vi "Process Feedback.vi"(8 "error in":errorcluster, 10 "Channel Feedback":T1, 11 "Sequence Executor in":refnum<class "Sequence Executor.lvclass">) -> (0 "error out":errorcluster, 3 "Sequence Executor out":refnum<class "Sequence Executor.lvclass">)   [LabVIEW 2026, in "Sequence Executor.lvclass"]
doc: "Handles one Channel Feedback from the rig. Stores Last Feedback; writes the Channel Values display (2-D string name | value | unit); if Running: latch Step Start ms on first feedback, Evaluate Step, and on done record the result and advance (Begin Step) or Finish Sequence."
uses:
  Sequence Executor.lvclass
  Sequence Executor.lvclass/Sequence Executor.ctl
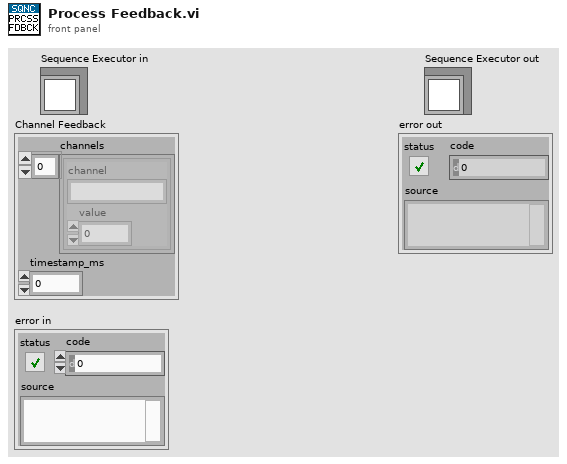
[diagram p1: front panel]
types:
  T1 = cluster{"channels":cluster{"channel":string, "value":dbl}[], "timestamp_ms":dbl}
  T2 = cluster{"step_no":i32, "step_name":string, "result":string, "reason":string, "measured":dbl, "target":dbl, "duration_ms":dbl}
  T3 = typedef "Rig Config.ctl" = cluster{"rig_id":string, "description":string, "plugin_class":string, "channels":T4[]}
  T4 = typedef "Channel Definition.ctl" = cluster{"name":string, "unit":string, "min":dbl, "max":dbl}
  T5 = typedef "Step Phase.ctl" = enum16{"Idle", "Settling", "Dwell", "Complete"}
  T6 = typedef "Sequence File.ctl" = cluster{"sequence_id":string, "description":string, "rig_config":string, "steps":T7[]}
  T7 = typedef "Step Config.ctl" = cluster{"step_no":i32, "step_name":string, "command_type":string, "setpoints":T8[], "conditions":T9[], "dwell_time_ms":i32, "timeout_ms":i32, "expected_result":string}
  T8 = typedef "Channel Value.ctl" = cluster{"channel":string, "value":dbl}
  T9 = typedef "Condition.ctl" = cluster{"channel":string, "target":dbl, "tolerance":dbl}
  T10 = typedef "Step Result.ctl" = cluster{"step_no":i32, "step_name":string, "result":string, "reason":string, "measured":dbl, "target":dbl, "duration_ms":dbl}
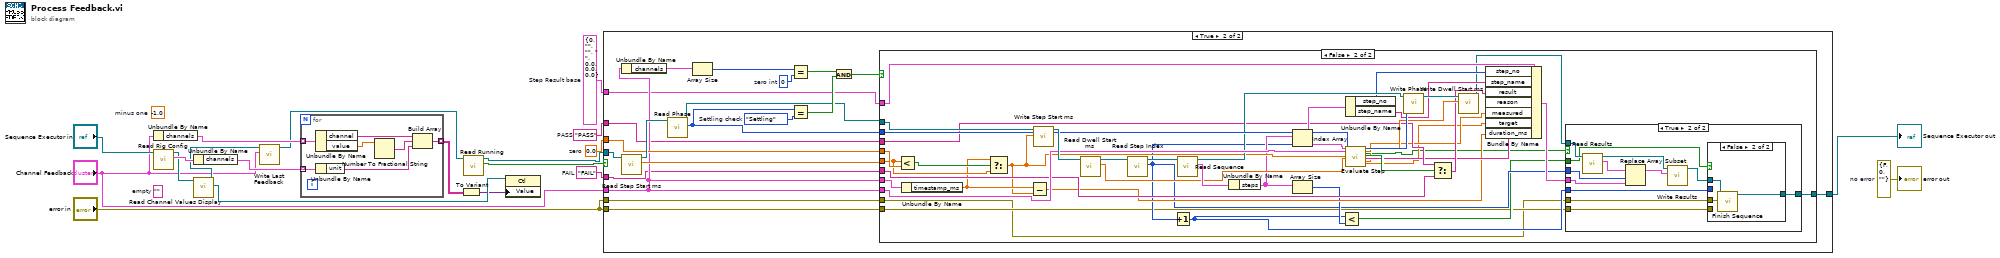
[diagram p0: block diagram]
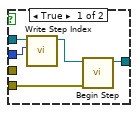
[diagram p5: hidden frame]
diagram:
  (unwired) -1.0  # minus one
  (unwired) ""  # empty
  w5 = T2 {"step_no"=0, "step_name"="", "result"="", "reason"=" ", "measured"=0.0, "target"=0.0, "duration_ms"=0.0}  # Step Result base
  w6 = "FAIL"  # FAIL
  w7 = "PASS"  # PASS
  w8 = 0.0  # zero
  w1 = errorcluster {"status"=FALSE, "code"=0, "source"=""}  # no error
  n1 = Unbundle By Name("Channel Feedback") -> ("channels"=w18:cluster{"channel":string, "value":dbl}[])
  n2 = call "Read Rig Config.vi"("Sequence Executor in"="Sequence Executor in") -> ("Rig Config"=w19:T3, "Sequence Executor out"=w16:refnum<class "Sequence Executor.lvclass">)  [unwired: 8 in, 1 out]
  n3 = Unbundle By Name(w19) -> ("channels"=w17:T4[])
  n4 = call "Read Channel Values Display.vi"("Sequence Executor in"=w16) -> ("Channel Values Display"=w14:refnum<vi>, "Sequence Executor out"=w12:refnum<class "Sequence Executor.lvclass">)  [unwired: 8 in, 1 out]
  n5 = call "Write Last Feedback.vi"("Channel Feedback"="Channel Feedback", "Sequence Executor in"=w12) -> ("Sequence Executor out"=w11:refnum<class "Sequence Executor.lvclass">)  [unwired: 8 in, 1 out]
  n6 = for {
    tunnel: w18 -> [w27] mode=indexing
    tunnel: w17 -> [w25] mode=indexing
    tunnel: [w21] -> w15 mode=indexing
    n7 = Unbundle By Name(w27) -> ("channel"=w24:string, "value"=w26:dbl)
    n8 = Unbundle By Name(w25) -> ("unit"=w22:string)
    n9 = Number To Fractional String(number=w26) -> (F-format string=w23:string)  [unwired: 3 in]
    n10 = Build Array(w24, w23, w22) -> (w21:string[])
  }
  n11 = To Variant(anything=w15) -> (Variant=w13:variant)
  n12 = call "Read Running.vi"("Sequence Executor in"=w11) -> ("Running"=w3:bool, "Sequence Executor out"=w10:refnum<class "Sequence Executor.lvclass">)  [unwired: 8 in, 1 out]
  n13 = property class="Ctl"(reference=w14, "Value"=w13) -> ()  [unwired: 1 in, 2 out]
  n14 = case shown="True" w3 {
    tunnel: w10 -> [w28 w48]
    tunnel: "Channel Feedback" -> [_ w36]
    tunnel: [w28 w29] -> w2
    tunnel: w8 -> [_ w37]
    tunnel: w7 -> [_ w35]
    tunnel: w6 -> [_ w34]
    tunnel: w5 -> [_ w33]
    tunnel: "error in" -> [_ w32]
    tunnel: "error in" -> [_ w31]
    frame False {
    }
    frame True {
      w43 = enum16{"Idle", "Settling", "Dwell", "Complete"}."Settling"  # Settling check
      w44 = 0  # zero int
      n15 = Unbundle By Name(w36) -> ("channels"=w46:cluster{"channel":string, "value":dbl}[])
      n16 = call "Read Step Start ms.vi"("Sequence Executor in"=w48) -> ("Step Start ms"=w39:dbl, "Sequence Executor out"=w47:refnum<class "Sequence Executor.lvclass">)  [unwired: 8 in, 1 out]
      n17 = call "Read Phase.vi"("Sequence Executor in"=w47) -> ("Step Phase"=w38:T5, "Sequence Executor out"=w40:refnum<class "Sequence Executor.lvclass">)  [unwired: 8 in, 1 out]
      n18 = Array Size(array=w46) -> (size(s)=w45:i32)
      n19 = Equal?(x=w45, y=w44) -> (x = y?=w42:bool)
      n20 = Equal?(x=w38, y=w43) -> (x = y?=w41:bool)
      n21 = And(x=w42, y=w41) -> (x .and. y?=w30:bool)
      n22 = case shown="False" w30 {
        tunnel: w40 -> [w49 w86]
        tunnel: w39 -> [_ w87]
        tunnel: w36 -> [_ w89]
        tunnel: w38 -> [_ w80]
        tunnel: [w49 w50] -> w29
        tunnel: w37 -> [_ w90]
        tunnel: w36 -> [_ w81]
        tunnel: w35 -> [_ w73]
        tunnel: w34 -> [_ w71]
        tunnel: w33 -> [_ w61]
        tunnel: w32 -> [_ w53]
        tunnel: w31 -> [_ w52]
        frame True {
        }
        frame False {
          n23 = Less?(x=w87, y=w90) -> (x < y?=w88:bool)
          n24 = Unbundle By Name(w89) -> ("timestamp_ms"=w70:dbl)
          n25 = Select(t=w70, s=w88, f=w87) -> (s? t:f=w69:dbl)
          n26 = Subtract(x=w70, y=w69) -> (x-y=w62:dbl)
          n27 = call "Write Step Start ms.vi"("Step Start ms"=w69, "Sequence Executor in"=w86) -> ("Sequence Executor out"=w85:refnum<class "Sequence Executor.lvclass">)  [unwired: 8 in, 1 out]
          n28 = call "Read Dwell Start ms.vi"("Sequence Executor in"=w85) -> ("Dwell Start ms"=w79:dbl, "Sequence Executor out"=w84:refnum<class "Sequence Executor.lvclass">)  [unwired: 8 in, 1 out]
          n29 = call "Read Step Index.vi"("Sequence Executor in"=w84) -> ("Step Index"=w56:i32, "Sequence Executor out"=w83:refnum<class "Sequence Executor.lvclass">)  [unwired: 8 in, 1 out]
          n30 = Increment(x=w56) -> (x+1=w55:i32)
          n31 = call "Read Sequence.vi"("Sequence Executor in"=w83) -> ("Sequence File"=w82:T6, "Sequence Executor out"=w78:refnum<class "Sequence Executor.lvclass">)  [unwired: 8 in, 1 out]
          n32 = Unbundle By Name(w82) -> ("steps"=w60:T7[])
          n33 = Index Array(array=w60, index=w56) -> (element=w74:T7)
          n34 = Array Size(array=w60) -> (size(s)=w59:i32)
          n35 = Less?(x=w55, y=w59) -> (x < y?=w54:bool)
          n36 = Unbundle By Name(w74) -> ("step_no"=w68:i32, "step_name"=w67:string)
          n37 = call "Evaluate Step.vi"("Step Config"=w74, "Channel Feedback"=w81, "Step Phase in"=w80, "step start ms"=w69, "dwell start ms"=w79) -> ("Step Phase out"=w77:T5, "dwell start ms out"=w75:dbl, "done"=w51:bool, "passed"=w72:bool, "reason"=w65:string, "measured"=w64:dbl, "target"=w63:dbl)  [unwired: 16 in]
          n38 = call "Write Phase.vi"("Step Phase"=w77, "Sequence Executor in"=w78) -> ("Sequence Executor out"=w76:refnum<class "Sequence Executor.lvclass">)  [unwired: 8 in, 1 out]
          n39 = Select(t=w73, s=w72, f=w71) -> (s? t:f=w66:string)
          n40 = call "Write Dwell Start ms.vi"("Dwell Start ms"=w75, "Sequence Executor in"=w76) -> ("Sequence Executor out"=w58:refnum<class "Sequence Executor.lvclass">)  [unwired: 8 in, 1 out]
          n41 = Bundle By Name(cluster=w61, "step_no"=w68, "step_name"=w67, "result"=w66, "reason"=w65, "measured"=w64, "target"=w63, "duration_ms"=w62) -> (w57:T2)
          n42 = case shown="True" w51 {
            tunnel: w58 -> [w91 w103]
            tunnel: w57 -> [_ w100]
            tunnel: w56 -> [_ w101]
            tunnel: w55 -> [_ w96]
            tunnel: w54 -> [_ w93]
            tunnel: [w91 w92] -> w50
            tunnel: w53 -> [_ w95]
            tunnel: w52 -> [_ w94]
            frame False {
            }
            frame True {
              n43 = call "Read Results.vi"("Sequence Executor in"=w103) -> ("Results"=w102:T10[], "Sequence Executor out"=w99:refnum<class "Sequence Executor.lvclass">)  [unwired: 8 in, 1 out]
              n44 = Replace Array Subset(array=w102, new element=w100, index=w101) -> (w98:T10[])
              n45 = call "Write Results.vi"("Results"=w98, "Sequence Executor in"=w99) -> ("Sequence Executor out"=w97:refnum<class "Sequence Executor.lvclass">)  [unwired: 8 in, 1 out]
              n46 = case shown="False" w93 {
                tunnel: w97 -> [w108 w111]
                tunnel: w96 -> [w107 _]
                tunnel: w95 -> [w105 _]
                tunnel: [w104 w109] -> w92
                tunnel: w94 -> [_ w110]
                frame True {
                  n47 = call "Write Step Index.vi"("Step Index"=w107, "Sequence Executor in"=w108) -> ("Sequence Executor out"=w106:refnum<class "Sequence Executor.lvclass">)  [unwired: 8 in, 1 out]
                  n48 = call "Begin Step.vi"("error in"=w105, "Sequence Executor in"=w106) -> ("Sequence Executor out"=w104:refnum<class "Sequence Executor.lvclass">)  [unwired: 8 in, 1 out]
                }
                frame False {
                  n49 = call "Finish Sequence.vi"("error in"=w110, "Sequence Executor in"=w111) -> ("Sequence Executor out"=w109:refnum<class "Sequence Executor.lvclass">)  [unwired: 8 in, 1 out]
                }
              }
            }
          }
        }
      }
    }
  }
  "Sequence Executor out" <- w2
  "error out" <- w1
